vi "Document Tests - .vi"(8 "error in (no error)":errorcluster) -> (0 "error out":errorcluster)   [LabVIEW 2017]
uses:
  <vilib>/addons/_JKI Toolkits/Caraya/classes/Test/Test.lvclass
  <vilib>/addons/_JKI Toolkits/Caraya/classes/Assert/Assert.lvclass
  <vilib>/addons/_JKI Toolkits/Caraya/classes/Assert/Assert Equal Value and Type_Variant.vi
  src/LabVIEW NPOI/Document/Document.lvclass
  <vilib>/addons/_JKI Toolkits/Caraya/classes/Assert/Assert Error.vi
  <vilib>/addons/_JKI Toolkits/Caraya/classes/Assert/Assert Not Error.vi
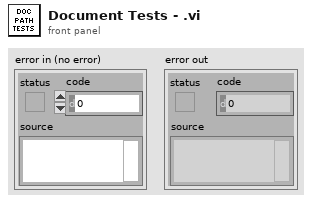
[diagram p1: front panel]
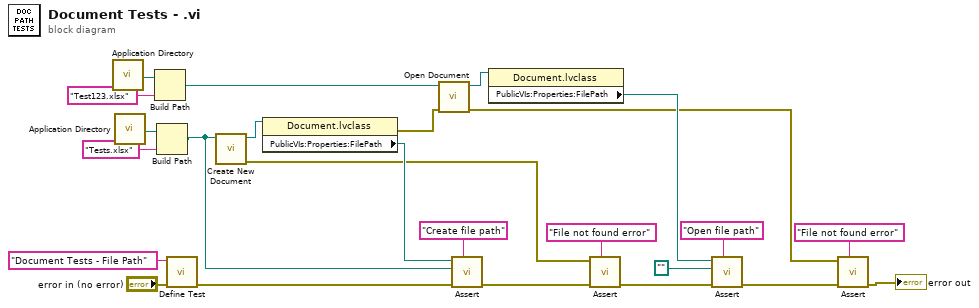
[diagram p0: block diagram]
diagram:
  n1 = call <vilib>:"Application Directory.vi"() -> ("Application Directory"=w19:path)
  n2 = call <vilib>:"Application Directory.vi"() -> ("Application Directory"=w2:path)
  n3 = Build Path(base path=w19, name or relative path="Test123.xlsx" ("Label")) -> (appended path=w5:path)
  n4 = Build Path(base path=w2, name or relative path="Tests.xlsx" ("Label")) -> (appended path=w1:path)
  n5 = call <vilib>:"Define Test.vi"("error in (no error)"="error in (no error)", "Label (VI Title)"="Document Tests - File Path") -> ("error out"=w22:errorcluster)  [unwired: 9 in]
  n6 = call "Create New Document.vi"("File Path"=w1) -> ("error out"=w7:errorcluster, "Document out"=w17:refnum<class "Document.lvclass">)  [unwired: 9 in]
  n7 = property on="Property Node" class="Document.lvclass"(reference=w17) -> (error out=w4:errorcluster, "PublicVIs:Properties:FilePath"=w14:path)  [unwired: 1 in, 1 out]
  n8 = call "Open Document.vi"("error in (no error)"=w4, "File Path"=w5) -> ("error out"=w8:errorcluster, "Document out"=w16:refnum<class "Document.lvclass">)  [unwired: 8 in]
  n9 = call-poly <vilib>:"Assert.vi"("Label"="Create file path", "error in (no error)"=w22, "Y"=w1, "X"=w14) -> ("error out"=w21:errorcluster)  [unwired: 7 in]
  n10 = property on="Property Node" class="Document.lvclass"(reference=w16) -> ("PublicVIs:Properties:FilePath"=w15:path)  [unwired: 1 in, 2 out]
  n11 = call-poly <vilib>:"Assert.vi"("Label"="File not found error", "error in (no error)"=w21, "Not Error?"=w7) -> ("error out"=w13:errorcluster)  [unwired: 8 in]
  n12 = call-poly <vilib>:"Assert.vi"("Label"="Open file path", "error in (no error)"=w13, "Y"=path "", "X"=w15) -> ("error out"=w11:errorcluster)  [unwired: 7 in]
  n13 = call-poly <vilib>:"Assert.vi"("Label"="File not found error", "error in (no error)"=w11, "Error?"=w8) -> ("error out"=→"error out":errorcluster)  [unwired: 8 in]
